vi "SPARK Get Analog Status.vi"   [LabVIEW 2027]
doc: "Get the periodic status of the analog sensor connected to the data port of the SPARK."
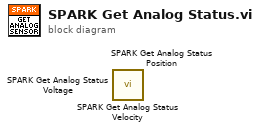
[diagram p0: block diagram]
diagram:
  n1 = call <vilib>:"SPARK Get Analog Status Velocity.vi"() -> ()  [unwired: 8 in, 4 out]
  n2 = call <vilib>:"SPARK Get Analog Status Position.vi"() -> ()  [unwired: 8 in, 4 out]
  n3 = call <vilib>:"SPARK Get Analog Status Voltage.vi"() -> ()  [unwired: 8 in, 4 out]
